vi "serial.vi"() -> ()   [LabVIEW 2017]
uses:
  <vilib>/Instr/_visa.llb/VISA Configure Serial Port (Instr).vi
panel:
  in  "PARAR":bool
  in  "PUERTO":refnum<visa-resource-name>="COM4"
  in  "Izquierda":bool
  in  "Derecha":bool
  in  "VELOCIDAD":dbl(knob) scale=0.0..100.0
  in  "LED2":bool
  in  "LED1":bool
  in  "stop":bool
  # "GIRO"
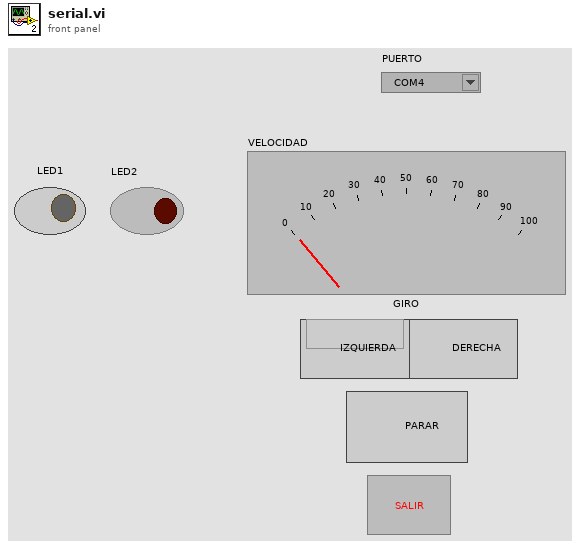
[diagram p1: front panel]
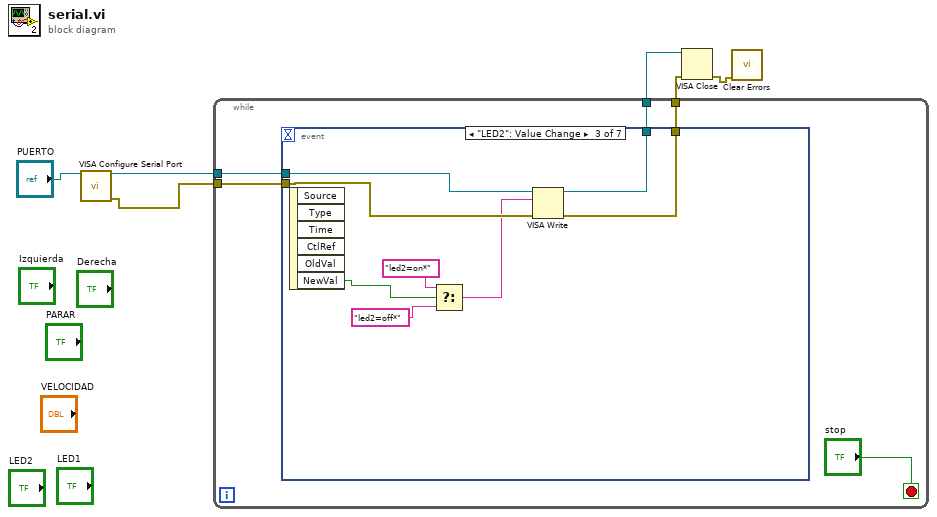
[diagram p0: block diagram]
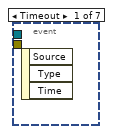
[diagram p2: hidden frame]
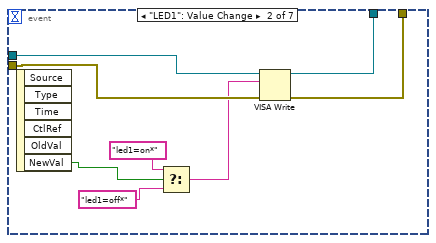
[diagram p3: hidden frame]
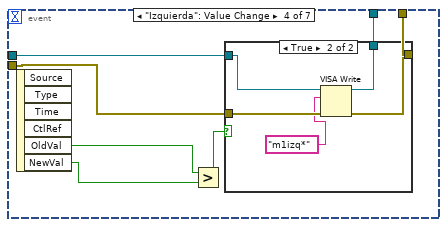
[diagram p4: hidden frame]
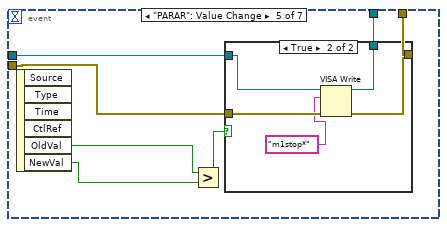
[diagram p6: hidden frame]
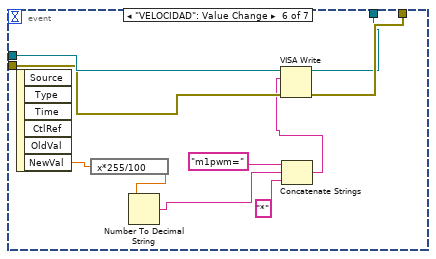
[diagram p8: hidden frame]
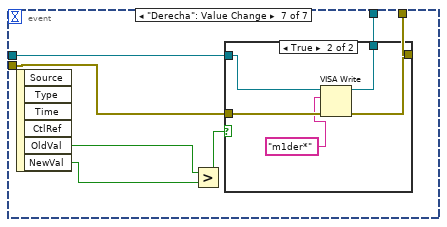
[diagram p9: hidden frame]
diagram:
  n1 = call-poly "VISA Configure Serial Port"("VISA resource name"="PUERTO") -> ("VISA resource name out"=w1:refnum<visa-resource-name>, "error out"=w2:errorcluster)  [unwired: 13 in]
  n2 = while {
    tunnel: w1 -> [w10]
    tunnel: w2 -> [w9]
    tunnel: [w8] -> w5
    tunnel: [w7] -> w4
    stop <- "stop" stop-if-true
    n3 = event shown="[2] \"LED2\": Value Change" {
      selector: _ -> [_ _ _ _ _ _ _]
      dyn-events: _ -> [_ _ _ _ _ _ _]
      timeout: _ -> [_ _ _ _ _ _ _]
      tunnel: w10 -> [_ w19 w27 w34 w46 w61 w68]
      tunnel: w9 -> [_ w18 w26 w33 w45 w60 w67]
      tunnel: [_ w13 w21 w32 w44 w58 w66] -> w8
      tunnel: [_ w12 w20 w31 w43 w59 w65] -> w7
      event Timeout {
        n4 = event-data() -> ()  [unwired: 1 in, 3 out]
      }
      event "LED1": Value Change {
        n5 = event-data() -> ("NewVal"=w17:bool)  [unwired: 1 in, 5 out]
        n6 = Select(t="led1=on*", s=w17, f="led1=off*") -> (s? t:f=w14:string)
        n7 = VISA Write(VISA resource name=w19, write buffer=w14, error in (no error)=w18) -> (VISA resource name out=w13:refnum<visa-resource-name>, error out=w12:errorcluster)  [unwired: 1 out]
      }
      event "LED2": Value Change {
        n8 = event-data() -> ("NewVal"=w25:bool)  [unwired: 1 in, 5 out]
        n9 = Select(t="led2=on*", s=w25, f="led2=off*") -> (s? t:f=w22:string)
        n10 = VISA Write(VISA resource name=w27, write buffer=w22, error in (no error)=w26) -> (VISA resource name out=w21:refnum<visa-resource-name>, error out=w20:errorcluster)  [unwired: 1 out]
      }
      event "Izquierda": Value Change {
        n11 = event-data() -> ("OldVal"=w30:bool, "NewVal"=w29:bool)  [unwired: 1 in, 4 out]
        n12 = Greater?(x=w30, y=w29) -> (0:w28:bool)
        n13 = case shown="True" w28 {
          tunnel: w34 -> [_ w39]
          tunnel: w33 -> [_ w38]
          tunnel: [_ w37] -> w32
          tunnel: [_ w36] -> w31
          frame False {
          }
          frame True {
            n14 = VISA Write(VISA resource name=w39, write buffer="m1izq*", error in (no error)=w38) -> (VISA resource name out=w37:refnum<visa-resource-name>, error out=w36:errorcluster)  [unwired: 1 out]
          }
        }
      }
      event "PARAR": Value Change {
        n15 = event-data() -> ("OldVal"=w42:bool, "NewVal"=w41:bool)  [unwired: 1 in, 4 out]
        n16 = Greater?(x=w42, y=w41) -> (0:w40:bool)
        n17 = case shown="True" w40 {
          tunnel: w46 -> [_ w51]
          tunnel: w45 -> [_ w50]
          tunnel: [_ w49] -> w44
          tunnel: [_ w48] -> w43
          frame False {
          }
          frame True {
            n18 = VISA Write(VISA resource name=w51, write buffer="m1stop*", error in (no error)=w50) -> (VISA resource name out=w49:refnum<visa-resource-name>, error out=w48:errorcluster)  [unwired: 1 out]
          }
        }
      }
      event "VELOCIDAD": Value Change {
        n19 = event-data() -> ("NewVal"=w53:dbl)  [unwired: 1 in, 5 out]
        n20 = expression code="x*255/100"(w53) -> (w52:dbl)
        n21 = Number To Decimal String(number=w52) -> (decimal integer string=w56:string)  [unwired: 1 in]
        n22 = Concatenate Strings("m1pwm=" ("string"), w56, "*" ("string")) -> (w54:string)
        n23 = VISA Write(VISA resource name=w61, write buffer=w54, error in (no error)=w60) -> (VISA resource name out=w58:refnum<visa-resource-name>, error out=w59:errorcluster)  [unwired: 1 out]
      }
      event "Derecha": Value Change {
        n24 = event-data() -> ("OldVal"=w64:bool, "NewVal"=w63:bool)  [unwired: 1 in, 4 out]
        n25 = Greater?(x=w64, y=w63) -> (0:w62:bool)
        n26 = case shown="True" w62 {
          tunnel: w68 -> [_ w73]
          tunnel: w67 -> [_ w72]
          tunnel: [_ w71] -> w66
          tunnel: [_ w70] -> w65
          frame False {
          }
          frame True {
            n27 = VISA Write(VISA resource name=w73, write buffer="m1der*", error in (no error)=w72) -> (VISA resource name out=w71:refnum<visa-resource-name>, error out=w70:errorcluster)  [unwired: 1 out]
          }
        }
      }
    }
  }
  n28 = VISA Close(VISA resource name=w5, error in (no error)=w4) -> (error out=w3:errorcluster)
  n29 = call <vilib>:"Clear Errors.vi"("error in (no error)"=w3) -> ()  [unwired: 5 in, 2 out]
